vi "Test To Report Entry.vi"(8 "error in (no error)":errorcluster, 9 "Asserts (aka. Test Cases)":T3[](array[typedef]), 10 "Node (aka. Test Suite)":T4, 11 "Test Report in":refnum<class "Test Report.lvclass">) -> (0 "error out":errorcluster, 2 "testsuite":T2, 3 "Test Report":refnum<class "Test Report.lvclass">, 4 "testcases extended":T1[](array[typedef]))   [LabVIEW 2020, in "Caraya.lvlib" / "Test Report.JUnit.lvclass"]
uses:
  Test Report.JUnit.lvclass
  Test Result/Test Node (Extended).ctl
  Test Result/Test Registration Data.ctl
  Test Result/Assert Event Data (Extended).ctl
  testsuite -- cluster.ctl
  extended -- cluster.ctl
  Test Report/Test Report.lvclass
  testcase -- cluster.ctl
  Test Result/Test Result.lvclass
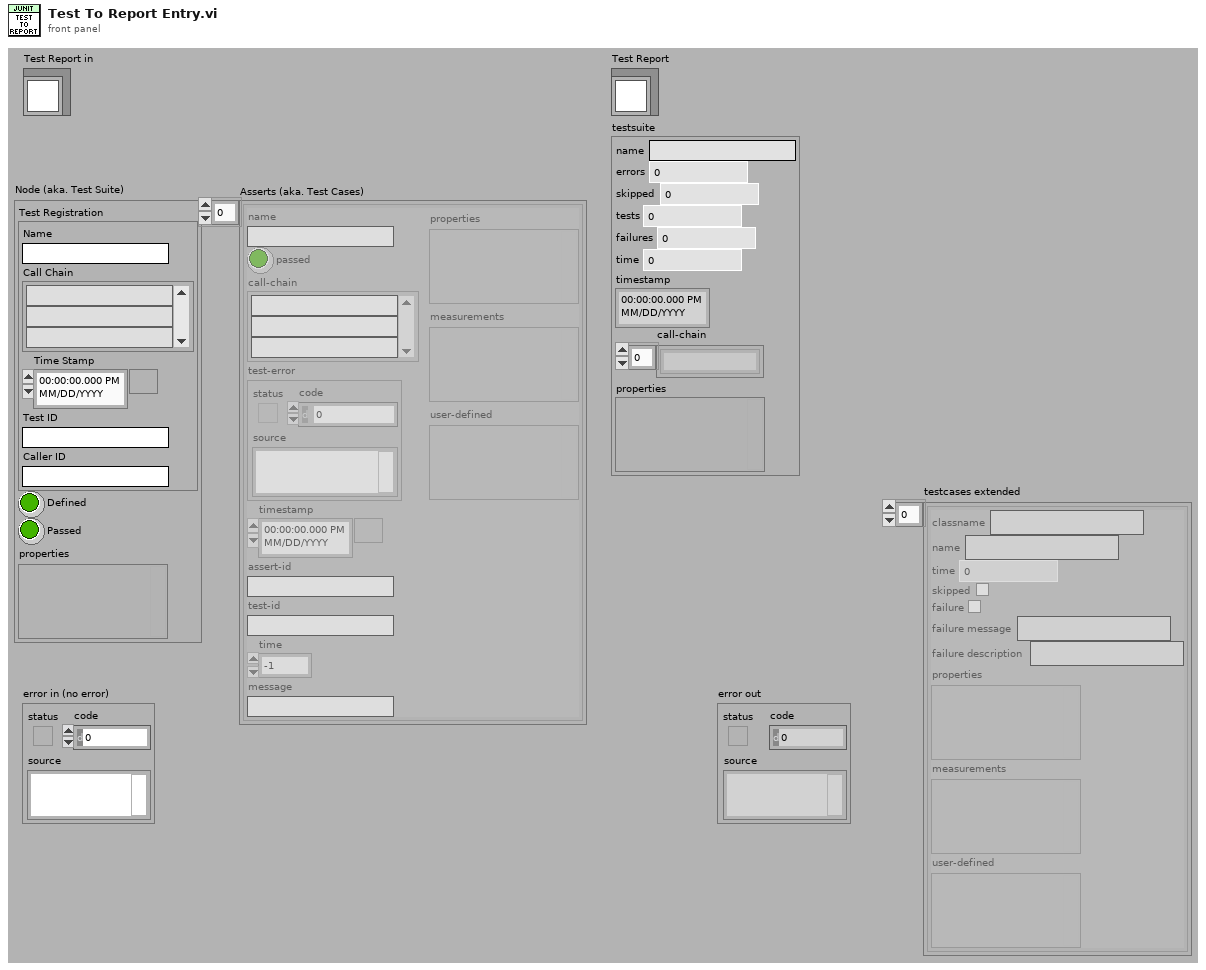
[diagram p1: front panel]
types:
  T1 = typedef "Caraya.lvlib/Test Report.JUnit.lvclass/extended -- cluster.ctl" = cluster{"classname":string, "name":string, "time":dbl, "skipped":bool, "failure":bool, "failure message":string, "failure description":string, "properties":variant, "measurements":variant, "user-defined":variant}
  T2 = typedef "Caraya.lvlib/Test Report.JUnit.lvclass/testsuite -- cluster.ctl" = cluster{"name":string, "errors":u32, "skipped":u32, "tests":u32, "failures":u32, "time":dbl, "timestamp":timestamp, "call-chain":string[], "properties":variant}
  T3 = typedef "Caraya.lvlib/Test Result.lvclass/Assert Event Data (Extended).ctl" = cluster{"name":string, "passed":bool, "call-chain":string[], "test-error":errorcluster, "timestamp":timestamp, "assert-id":string, "test-id":string, "time":dbl, "message":string, "properties":variant, "measurements":variant, "user-defined":variant}
  T4 = typedef "Caraya.lvlib/Test Result.lvclass/Test Node (Extended).ctl" = cluster{"Test Registration":T5, "Defined":bool, "Passed":bool, "properties":variant}
  T5 = typedef "Caraya.lvlib/Test Result.lvclass/Test Registration Data.ctl" = cluster{"Name":string, "Call Chain":string[], "Time Stamp":timestamp, "Test ID":string, "Caller ID":string}
  T6 = typedef "Caraya.lvlib/Test Report.JUnit.lvclass/testcase -- cluster.ctl" = cluster{"classname":string, "name":string, "time":dbl, "skipped":bool, "failure":bool, "failure message":string, "failure description":string}
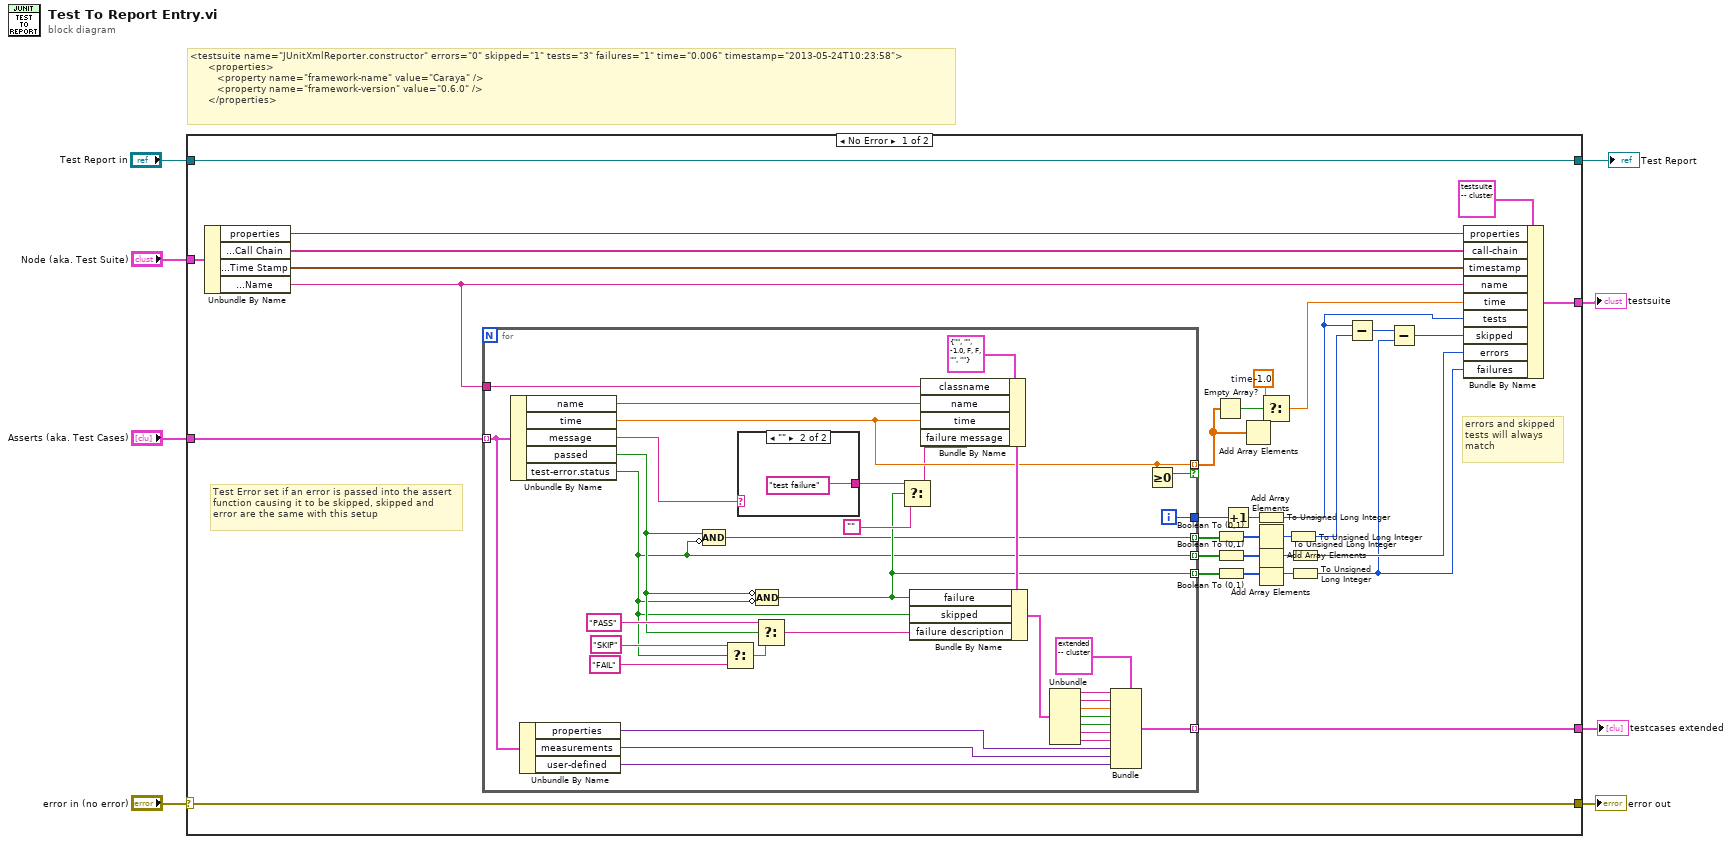
[diagram p0: block diagram]
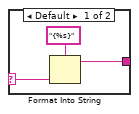
[diagram p2: hidden frame]
diagram:
  # "<testsuite name=\"JUnitXmlReporter.constructor\" errors=\"0\" skipped=\"1\" tests=\"3\" failures=\"1\" time=\"0.006\" timestamp=\"2013-05-24T10:23:58\">\n      <properties>\n         <property name=\"framework-name\" value=\"Caraya\" />\n         <property name=\"framework-version\" value=\"0.6.0\" />\n      </properties>"
  n1 = case shown="No Error" "error in (no error)" {
    selector: "error in (no error)" -> [w40 w81]
    tunnel: [w40 w81] -> w7
    tunnel: "Node (aka. Test Suite)" -> [w41 _]
    tunnel: "Asserts (aka. Test Cases)" -> [w39 _]
    tunnel: [w36 _] -> w2
    tunnel: [w11 _] -> w1
    tunnel: "Test Report in" -> [w9 w80]
    tunnel: [w9 w80] -> w3
    frame No Error {
      w27 = -1.0  # time
      # "errors and skipped\ntests will always\nmatch"
      # "Test Error set if an error is passed into the assert\nfunction causing it to be skipped, skipped and \nerror are the same with this setup"
      n2 = Unbundle By Name(w41) -> ("properties"=w10:variant, "Test Registration.Call Chain"=w19:string[], "Test Registration.Time Stamp"=w24:timestamp, "Test Registration.Name"=w18:string)
      n3 = for {
        tunnel: w39 -> [w55] mode=indexing
        tunnel: [w56] -> w38 mode=indexing
        tunnel: [w57] -> w33 mode=indexing
        tunnel: w18 -> [w68]
        tunnel: [w64] -> w29 mode=indexing if=w71
        tunnel: [w69] -> w25
        tunnel: [w59] -> w15 mode=indexing
        tunnel: [w42] -> w11 mode=indexing
        i -> [w69]
        n4 = Unbundle By Name(w55) -> ("name"=w65:string, "time"=w64:dbl, "message"=w60:string, "passed"=w58:bool, "test-error.status"=w57:bool)
        n5 = Unbundle By Name(w55) -> ("properties"=w45:variant, "measurements"=w44:variant, "user-defined"=w43:variant)
        n6 = Compound Arithmetic op=AND(w58, invert w57) -> (w56:bool)
        n7 = Select(t="SKIP" ("failure message"), s=w57, f="FAIL" ("failure message")) -> (s? t:f=w74:string)
        n8 = case shown="\"\"" w60 {
          selector: w60 -> [w76 _]
          tunnel: [w77 "test failure" ("failure message")] -> w61
          frame Default {
            n9 = Format Into String(format string="{%s}", w76) -> (resulting string=w77:string)  [unwired: 2 in, 1 out]
          }
          frame "" {
          }
        }
        n10 = Compound Arithmetic op=AND(invert w58, invert w57) -> (w59:bool)
        n11 = Select(t="PASS" ("failure message"), s=w58, f=w74) -> (s? t:f=w70:string)
        n12 = Select(t=w61, s=w59, f="") -> (s? t:f=w62:string)
        n13 = Bundle By Name(cluster=T6 {"classname"="", "name"="", "time"=-1.0, "skipped"=FALSE, "failure"=FALSE, "failure message"="", "failure description"=""} ("testcase"), "classname"=w68, "name"=w65, "time"=w64, "failure message"=w62) -> (w66:T6)
        n14 = Bundle By Name(cluster=w66, "failure"=w59, "skipped"=w57, "failure description"=w70) -> (w53:T6)
        n15 = Unbundle(w53) -> ("classname"=w54:string, "name"=w52:string, "time"=w46:dbl, "skipped"=w47:bool, "failure"=w48:bool, "failure message"=w49:string, "failure description"=w50:string)
        n16 = Bundle(cluster=T1 {"classname"="", "name"="", "time"=0.0, "skipped"=FALSE, "failure"=FALSE, "failure message"="", "failure description"="", "properties"=variant, "measurements"=variant, "user-defined"=variant} ("testcase"), "classname"=w54, "name"=w52, "time"=w46, "skipped"=w47, "failure"=w48, "failure message"=w49, "failure description"=w50, "properties"=w45, "measurements"=w44, "user-defined"=w43) -> (w42:T1)
        n17 = Greater Or Equal To 0?(x=w64) -> (x >= 0?=w71:bool)
      }
      n18 = Empty Array?(array=w29) -> (empty?=w28:bool)
      n19 = Boolean To (0,1)(Boolean=w38) -> (0, 1=w37:i16[])
      n20 = Boolean To (0,1)(Boolean=w33) -> (0, 1=w34:i16[])
      n21 = Boolean To (0,1)(Boolean=w15) -> (0, 1=w16:i16[])
      n22 = Increment(x=w25) -> (x+1=w21:i32)
      n23 = Add Array Elements(numeric array=w29) -> (sum=w26:dbl)
      n24 = To Unsigned Long Integer(number=w21) -> (unsigned 32bit integer=w20:u32)
      n25 = Add Array Elements(numeric array=w37) -> (sum=w35:i16)
      n26 = Add Array Elements(numeric array=w34) -> (sum=w32:i16)
      n27 = Add Array Elements(numeric array=w16) -> (sum=w17:i16)
      n28 = Select(t=w27, s=w28, f=w26) -> (s? t:f=w23:dbl)
      n29 = To Unsigned Long Integer(number=w35) -> (unsigned 32bit integer=w31:u32)
      n30 = To Unsigned Long Integer(number=w32) -> (unsigned 32bit integer=w30:u32)
      n31 = To Unsigned Long Integer(number=w17) -> (unsigned 32bit integer=w14:u32)
      n32 = Subtract(x=w20, y=w31) -> (x-y=w12:u32)
      n33 = Subtract(x=w12, y=w14) -> (x-y=w13:u32)
      n34 = Bundle By Name(cluster=T2 {"name"="", "errors"=0, "skipped"=0, "tests"=0, "failures"=0, "time"=-1.0, "timestamp"=timestamp(0 s since 1904-01-01), "call-chain"=[], "properties"=variant} ("testsuite"), "properties"=w10, "call-chain"=w19, "timestamp"=w24, "name"=w18, "time"=w23, "tests"=w20, "skipped"=w13, "errors"=w30, "failures"=w14) -> (w36:T2)
    }
    frame Error {
    }
  }
  "error out" <- w7
  "testsuite" <- w2
  "testcases extended" <- w1
  "Test Report" <- w3
